vi "user32 GetWindowRect.vi"(0 "hWnd":u64, 11 "error in":errorcluster) -> (4 "RECT":T1, 6 "return value":i32, 15 "error out":errorcluster)   [LabVIEW 2020, in "RemoteVI.lvlib"]
doc: "Returns the bounding rectangle of the window hWnd in SCREEN coordinates through user32.dll GetWindowRect (stdcall, called in any thread). The rectangle travels to the DLL as a RECT {LONG left, top, right, bottom}; right and bottom are exclusive. return value is the Win32 BOOL: non-zero on success. When error in carries an error the DLL is not called. Generated by scripts\\Build Win32 Wrappers.vi - do not edit by hand, rebuild it."
uses:
  RemoteVI.lvlib
  user32.dll
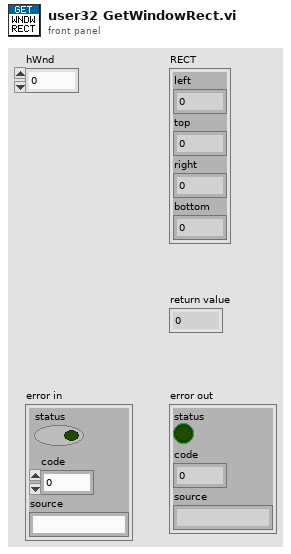
[diagram p1: front panel]
types:
  T1 = cluster{"left":i32, "top":i32, "right":i32, "bottom":i32}
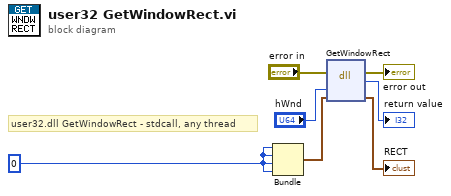
[diagram p0: block diagram]
diagram:
  w7 = 0
  # "user32.dll GetWindowRect - stdcall, any thread"
  n1 = Bundle(w7, w7, w7, w7) -> (w2:cluster{i32, i32, i32, i32})  [unwired: 1 in]
  n2 = dll-call lib="user32.dll" fn="GetWindowRect"(error in="error in", "hWnd"="hWnd", "lpRect"=w2) -> (error out=→"error out":errorcluster, →"return value":i32, "lpRect"=→"RECT":cluster{i32, i32, i32, i32})  [unwired: 3 in, 1 out]
